vi "MAPS.vi"() -> ()   [LabVIEW 2025]
uses:
  States.ctl
panel:
  out "Trackfile generation":bool
  out "Route waypoints coordinates":string
  in  "stop":bool
  out "GPS signal generation":bool
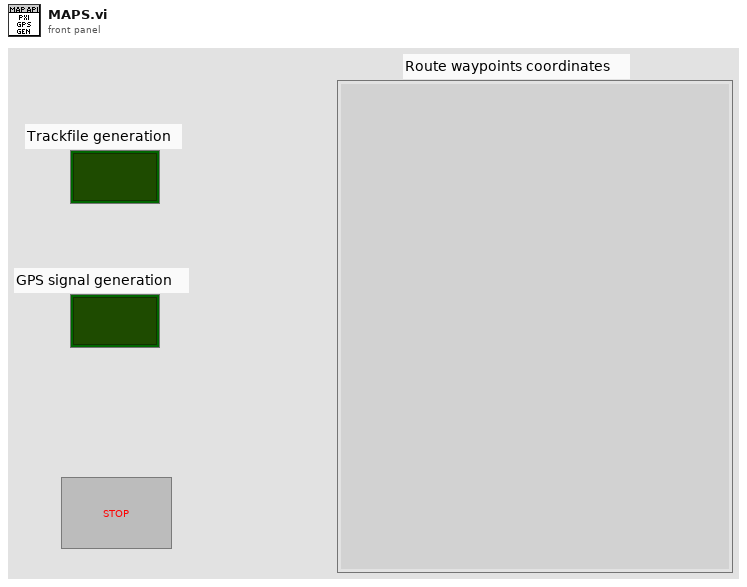
[diagram p1: front panel]
types:
  T1 = typedef "States.ctl" = enum16{"NOP", "StartGeneration", "GenerateTrajFile"}
  T2 = enum16{"open", "replace", "create", "open or create", "replace or create", "replace or create with confirmation"}
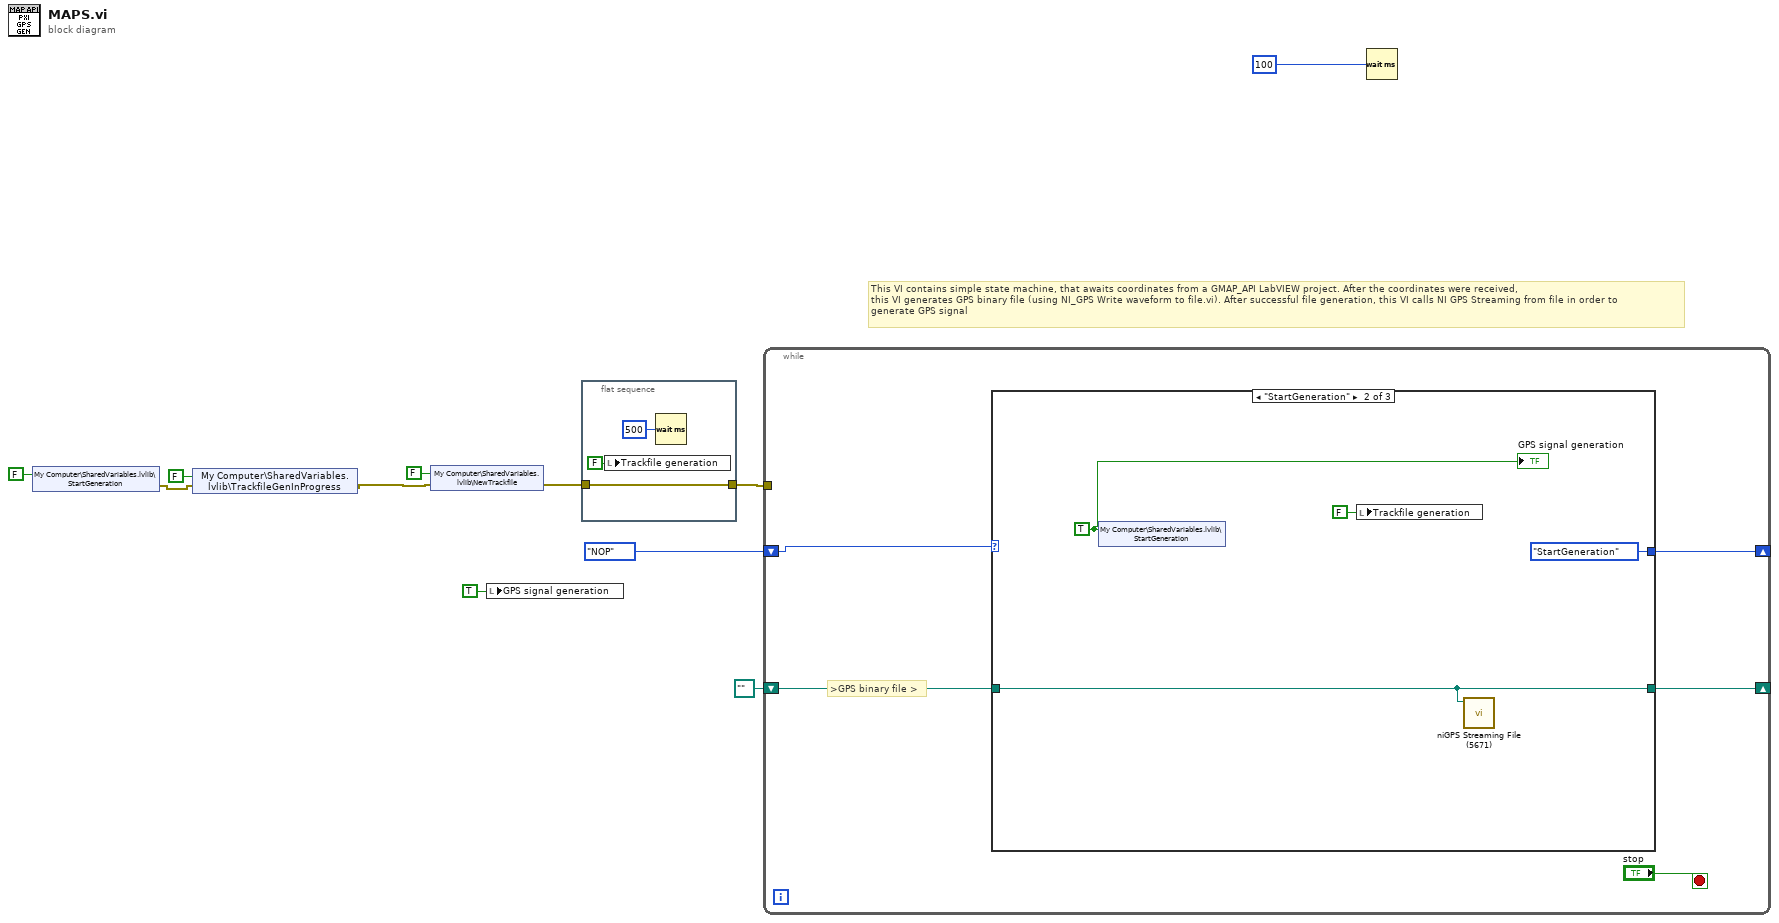
[diagram p0: block diagram]
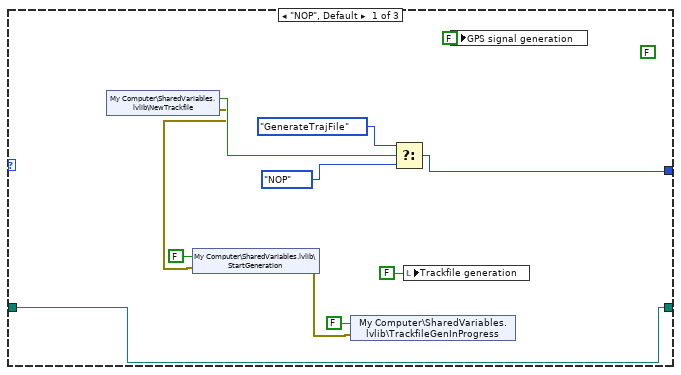
[diagram p2: hidden frame]
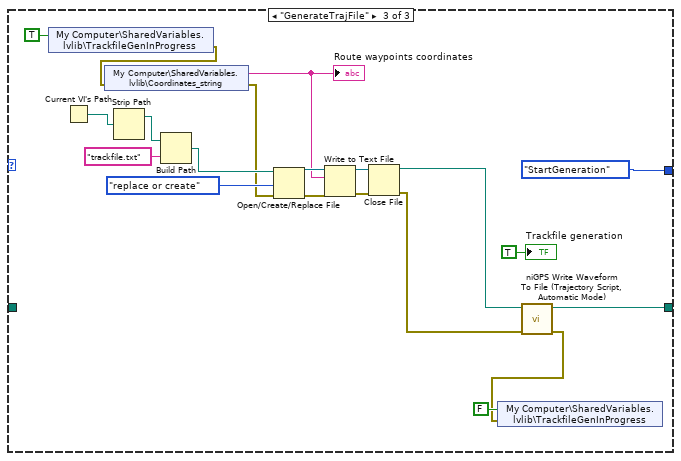
[diagram p3: hidden frame]
diagram:
  # "This VI contains simple state machine, that awaits coordinates from a GMAP_API LabVIEW project. After the coordinates were received,\nthis VI generates GPS binary file (using NI_GPS Write waveform to file.vi). After successful file generation, this VI calls NI GPS Streaming from file in order to\ngenerate GPS signal"
  n1 = shared-variable "My Computer\\SharedVariables.lvlib\\StartGeneration"(FALSE ("StartGeneration")) -> (error out=w5:errorcluster)  [unwired: 1 in]
  n2 = shared-variable "My Computer\\SharedVariables.lvlib\\TrackfileGenInProgress"(FALSE ("TrackfileGenInProgress"), error in=w5) -> (error out=w7:errorcluster)
  n3 = shared-variable "My Computer\\SharedVariables.lvlib\\NewTrackfile"(FALSE ("NewTrackfile"), error in=w7) -> (error out=w3:errorcluster)
  n4 = local write "GPS signal generation"(TRUE ("GPS signal generation")) -> ()
  n5 = flat-sequence {
    tunnel: [w14] -> w4
    tunnel: w3 -> [w14]
    frame #0 {
      n6 = local write "Trackfile generation"(FALSE ("TrackfileGeneration")) -> ()
      n7 = Wait (ms)(milliseconds to wait=u32 500) -> ()  [unwired: 1 out]
    }
  }
  n8 = while {
    shift-right: [w17] -> _
    shift-left: States."NOP" -> [w18]
    tunnel: w4 -> [_]
    shift-right: [w16] -> _
    shift-left: path "" ("Output GPS Binary File Path 2") -> [w15]
    stop <- "stop" stop-if-true
    # ">GPS binary file >"
    n9 = case shown="\"StartGeneration\"" w18 {
      tunnel: [w27 States."StartGeneration" States."StartGeneration"] -> w17
      tunnel: [w21 w33 w36] -> w16
      tunnel: w15 -> [w21 w33 _]
      frame "NOP", Default {
        (unwired) FALSE ("StartGeneration")
        n10 = shared-variable "My Computer\\SharedVariables.lvlib\\NewTrackfile"() -> (w30:bool, error out=w24:errorcluster)  [unwired: 1 in]
        n11 = shared-variable "My Computer\\SharedVariables.lvlib\\StartGeneration"(FALSE ("StartGeneration"), error in=w24) -> (error out=w23:errorcluster)
        n12 = shared-variable "My Computer\\SharedVariables.lvlib\\TrackfileGenInProgress"(FALSE ("TrackfileGenInProgress"), error in=w23) -> ()  [unwired: 1 out]
        n13 = Select(t=States."GenerateTrajFile", s=w30, f=States."NOP") -> (s? t:f=w27:T1)
        n14 = local write "Trackfile generation"(FALSE ("TrackfileGeneration")) -> ()
        n15 = local write "GPS signal generation"(FALSE ("StartGeneration")) -> ()
      }
      frame "StartGeneration" {
        w32 = TRUE ("StartGeneration")
        n16 = shared-variable "My Computer\\SharedVariables.lvlib\\StartGeneration"(w32) -> ()  [unwired: 1 in, 1 out]
        n17 = local write "Trackfile generation"(FALSE ("TrackfileGeneration")) -> ()
        n18 = call "niGPS Streaming File (5671).vi"("GPS Binary File Path"=w33) -> ()  [unwired: 9 in]
        "GPS signal generation" <- w32
      }
      frame "GenerateTrajFile" {
        n19 = shared-variable "My Computer\\SharedVariables.lvlib\\TrackfileGenInProgress"(TRUE ("TrackfileGenInProgress")) -> (error out=w54:errorcluster)  [unwired: 1 in]
        n20 = Current VI's Path() -> (path=w38:path)
        n21 = shared-variable "My Computer\\SharedVariables.lvlib\\Coordinates_string"(error in=w54) -> (w44:string, error out=w47:errorcluster)
        "Route waypoints coordinates" <- w44
        n22 = Strip Path(path=w38) -> (stripped path=w37:path)  [unwired: 1 out]
        n23 = Build Path(base path=w37, name or relative path="trackfile.txt") -> (appended path=w49:path)
        n24 = Open/Create/Replace File(file path (use dialog)=w49, error in=w47, operation (0:open)=T2."replace or create") -> (refnum out=w45:refnum<file>, error out=w46:errorcluster)  [unwired: 3 in, 1 out]
        n25 = Write to Text File(file (use dialog)=w45, text=w44, error in=w46) -> (refnum out=w42:refnum<file>, error out=w43:errorcluster)  [unwired: 1 in, 1 out]
        n26 = Close File(refnum=w42, error in=w43) -> (path=w41:path, error out=w40:errorcluster)
        n27 = call "niGPS Write Waveform To File (Trajectory Script, Automatic Mode).vi"("error in"=w40, "Motion File Path"=w41) -> ("Error Out"=w51:errorcluster, "Output GPS Binary File Path 2"=w36:path)  [unwired: 6 in]
        n28 = shared-variable "My Computer\\SharedVariables.lvlib\\TrackfileGenInProgress"(FALSE ("TrackfileGenInProgress"), error in=w51) -> ()  [unwired: 1 out]
        "Trackfile generation" <- TRUE ("TrackfileGeneration")
      }
    }
  }
  n29 = Wait (ms)(milliseconds to wait=u32 100) -> ()  [unwired: 1 out]
